vi "Open.vi"(10 "Lancer server.py":string="\"D:\\Home\\eschaub\\Documents\\INFORMATIQUE\\LabVIEW-Python TCP\\Public repo\\Python\\lancer_serveur.py\"", 11 "port":u16=5000) -> (0 "error out":errorcluster, 3 "connection ID":refnum<k5>)   [LabVIEW 2020, in "LabVIEW-Python TCP Lib.lvlib"]
uses:
  LabVIEW-Python TCP Lib.lvlib
panel:
  out "code":i32
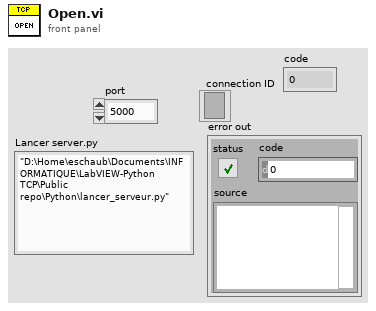
[diagram p1: front panel]
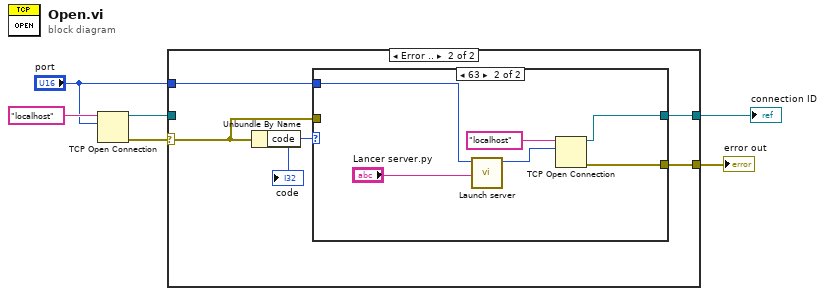
[diagram p0: block diagram]
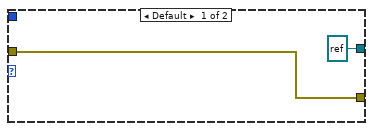
[diagram p3: hidden frame]
diagram:
  n1 = TCP Open Connection(address="localhost", remote port or service name="port") -> (connection ID=w4:refnum<k5>, error out=w5:errorcluster)  [unwired: 3 in]
  n2 = case shown="Error .." w5 {
    selector: w5 -> [w7 w9]
    tunnel: w4 -> [w8 _]
    tunnel: [w8 w11] -> w3
    tunnel: "port" -> [_ w12]
    tunnel: [w7 w10] -> w1
    frame No Error {
    }
    frame Error {
      n3 = Unbundle By Name(w9) -> ("code"=w13:i32)
      "code" <- w13
      n4 = case shown="63" w13 {
        tunnel: w12 -> [_ w18]
        tunnel: [refnum<k5> refnum ("connection ID") w17] -> w11
        tunnel: [w14 w16] -> w10
        tunnel: w9 -> [w14 _]
        frame Default {
        }
        frame 63 {
          n5 = call "Launch server.vi"("Lancer server.py"="Lancer server.py", "Port"=w18) -> ("Port out"=w19:u16)  [unwired: 9 in]
          n6 = TCP Open Connection(address="localhost", remote port or service name=w19) -> (connection ID=w17:refnum<k5>, error out=w16:errorcluster)  [unwired: 3 in]
        }
      }
    }
  }
  "connection ID" <- w3
  "error out" <- w1
